vi "Publish Random Event.vi"(11 "market":T1) -> (3 "market out":T1)   [LabVIEW 2020, in "Full Featured MCP Server.lvlib"]
doc: "About once every 50 seconds picks a random stock and a random event from the Event Catalogue and applies it. Strong companies get good news more often and weak companies bad news (Good Outcome.vi), so the news mostly agree with the quality of a company, but not always. The size of each event varies."
uses:
  Full Featured MCP Server.lvlib
  Market State.ctl
  News Item.ctl
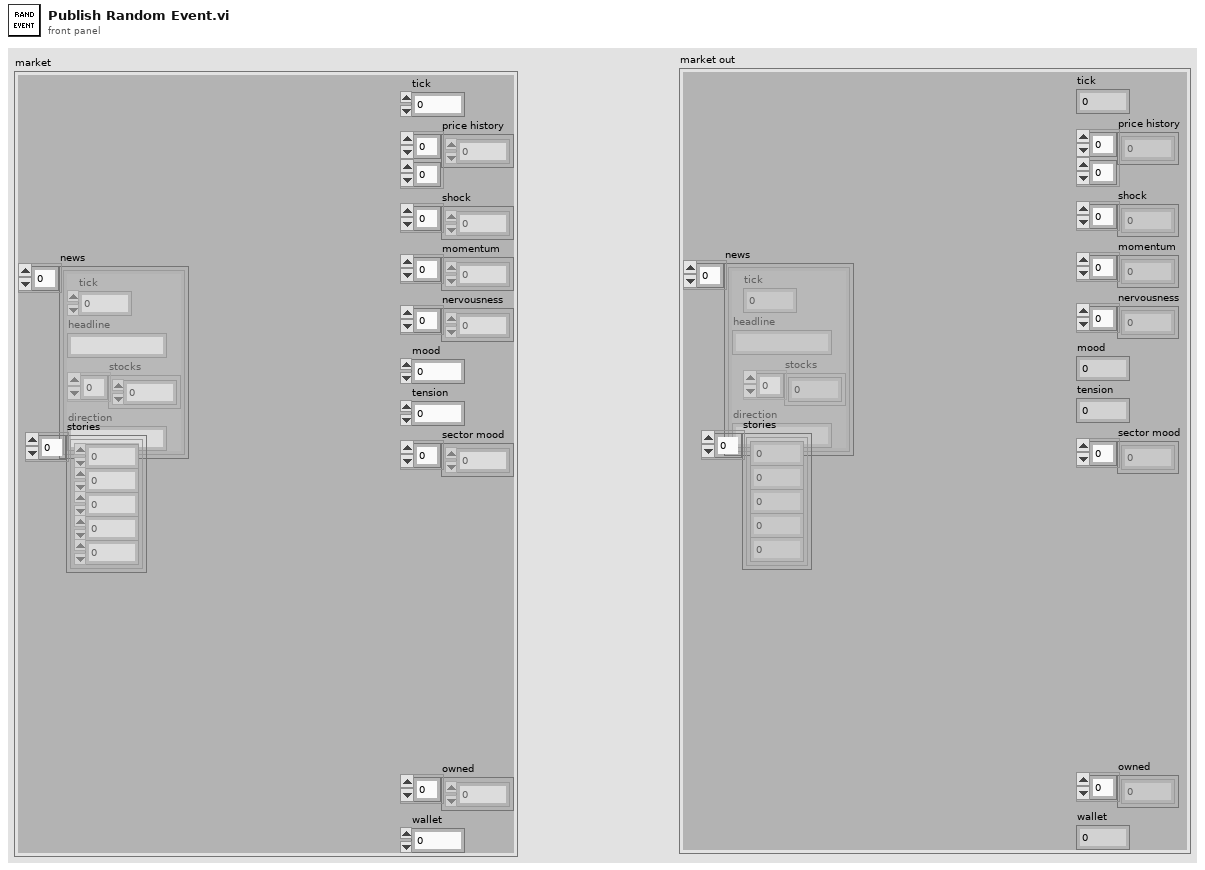
[diagram p1: front panel]
types:
  T1 = typedef "Full Featured MCP Server.lvlib/Market State.ctl" = cluster{"tick":i32, "price history":dbl[][], "shock":dbl[], "momentum":dbl[], "nervousness":dbl[], "mood":dbl, "tension":dbl, "sector mood":dbl[], "news":T2[], "stories":cluster{"arc":i32, "step":i32, "due":i32, "stock":i32, "other":i32}[], "owned":i32[], "wallet":dbl}
  T2 = typedef "Full Featured MCP Server.lvlib/News Item.ctl" = cluster{"tick":i32, "headline":string, "stocks":i32[], "direction":string}
  T3 = cluster{"headline":string, "scope":enum16{"one stock", "two stocks", "sector", "market"}, "direction":string, "jump":dbl, "follow":dbl, "jump other":dbl, "follow other":dbl}[]
  T4 = cluster{"headline":string, "scope":enum16{"one stock", "two stocks", "sector", "market"}, "direction":string, "jump":dbl, "follow":dbl, "jump other":dbl, "follow other":dbl}
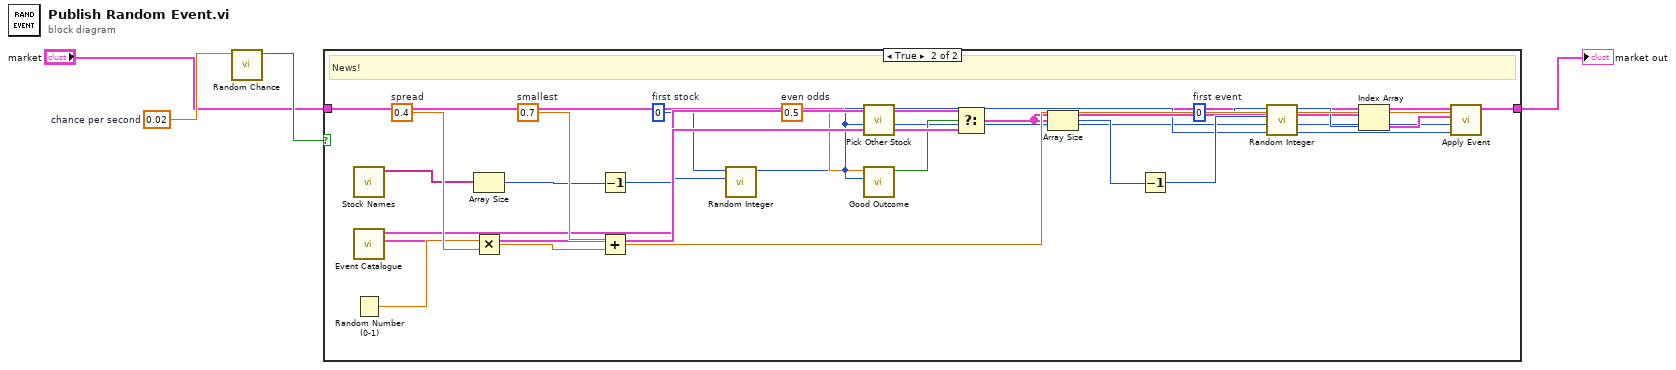
[diagram p0: block diagram]
diagram:
  w2 = 0.02  # chance per second
  n1 = call "Random Chance.vi"("probability"=w2) -> ("happened?"=w3:bool)  [unwired: 10 in]
  n2 = case shown="True" w3 {
    tunnel: "market" -> [w5 w6]
    tunnel: [w5 w7] -> w4
    frame False {
      # "Nothing happens"
    }
    frame True {
      w26 = 0.4  # spread
      w24 = 0.7  # smallest
      w19 = 0  # first event
      w14 = 0.5  # even odds
      w10 = 0  # first stock
      # "News!"
      n3 = call "Stock Names.vi"() -> ("names"=w8:string[])  [unwired: 11 in]
      n4 = call "Event Catalogue.vi"() -> ("bad news"=w17:T3, "good news"=w16:T3)  [unwired: 8 in, 2 out]
      n5 = Random Number (0-1)() -> (number: 0 to 1=w25:dbl)
      n6 = Array Size(array=w8) -> (size(s)=w9:i32)
      n7 = Multiply(x=w25, y=w26) -> (x*y=w27:dbl)
      n8 = Decrement(x=w9) -> (x-1=w11:i32)
      n9 = Add(x=w24, y=w27) -> (x+y=w28:dbl)
      n10 = call "Random Integer.vi"("high"=w11, "low"=w10) -> ("number"=w12:i32)  [unwired: 9 in]
      n11 = call "Pick Other Stock.vi"("stock"=w12) -> ("other"=w13:i32)  [unwired: 10 in]
      n12 = call "Good Outcome.vi"("stock"=w12, "odds"=w14) -> ("good?"=w15:bool)  [unwired: 9 in]
      n13 = Select(t=w16, s=w15, f=w17) -> (s? t:f=w18:T3)
      n14 = Array Size(array=w18) -> (size(s)=w20:i32)
      n15 = Decrement(x=w20) -> (x-1=w21:i32)
      n16 = call "Random Integer.vi"("high"=w21, "low"=w19) -> ("number"=w22:i32)  [unwired: 9 in]
      n17 = Index Array(array=w18, index=w22) -> (element=w23:T4)
      n18 = call "Apply Event.vi"("scale"=w28, "other"=w13, "stock"=w12, "event"=w23, "market"=w6) -> ("market out"=w7:T1)  [unwired: 6 in]
    }
  }
  "market out" <- w4
